vi "GetFormattedStringBounds.vi"(0 "reference":refnum<class "MultiLineString.lvclass">, 1 "graphics":refnum<class "Graphics.lvclass">, 5 "error in (no error)":errorcluster, 6 "TargetBounds(IgnoreIfZero)":T1 {"height" format="%.2f"; "width" format="%.2f"; "y" format="%.2f"; "x" format="%.2f"}) -> (14 "reference out":refnum<class "MultiLineString.lvclass">, 15 "bounds":T1 {"height" format="%.2f"; "width" format="%.2f"; "y" format="%.2f"; "x" format="%.2f"}, 19 "error out":errorcluster)   [LabVIEW 2020, in "MultiLineString.lvclass"]
doc: "public Rectangle2D getBounds(Graphics2D g2)"
uses:
  <resource>/Framework/Providers/Open_GDS/UML/MultiLineString_class/MultiLineString.lvclass
  <resource>/Framework/Providers/Open_GDS/UML/General/Rectangle/Rectangle Rectangle2D.ctl
  <resource>/Framework/Providers/Open_GDS/UML/Graphics_class/Graphics.lvclass
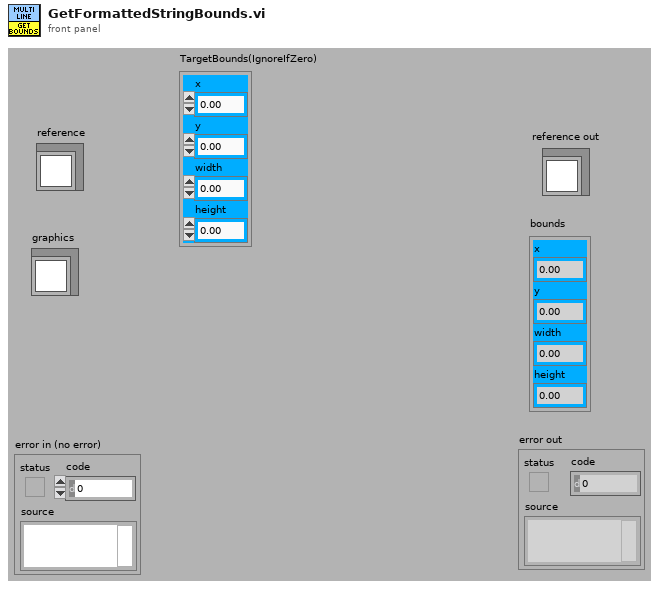
[diagram p1: front panel]
types:
  T1 = typedef "Rectangle Rectangle2D.ctl" = cluster{"x":dbl, "y":dbl, "width":dbl, "height":dbl}
  T2 = typedef "MultiLineString.lvclass/ObjectAttributes.ctl" = cluster{"GAP":i32, "text":string, "justification":T3, "size":T4, "underlined":bool}
  T3 = typedef "MultiLineString.lvclass/JustificationType.ctl" = enum16{"LEFT", "CENTER", "RIGHT"}
  T4 = typedef "MultiLineString.lvclass/SizeType.ctl" = enum16{"LARGE", "NORMAL", "SMALL"}
  T5 = typedef "Graphics.lvclass/FontType.ctl" = cluster{"Font Name:":string, "Size":i16, "Strikeout?":bool, "Italic?":bool, "Underline?":bool, "Outline?":bool, "Shadow?":bool, "Bold?":bool}
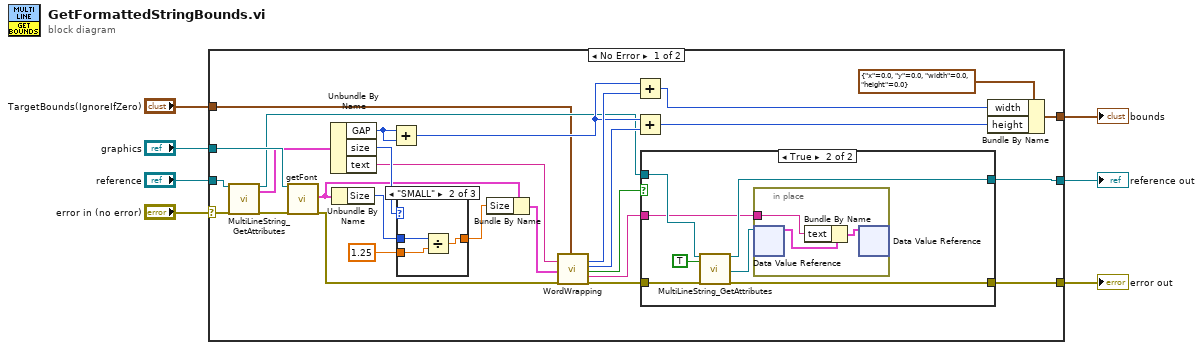
[diagram p0: block diagram]
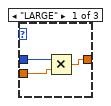
[diagram p3: hidden frame]
diagram:
  n1 = case shown="No Error" "error in (no error)" {
    selector: "error in (no error)" -> [w32 w55]
    tunnel: "reference" -> [w35 w56]
    tunnel: [w13 w55] -> w6
    tunnel: [w12 w56] -> w5
    tunnel: [w34 _] -> w3
    tunnel: "graphics" -> [w33 _]
    tunnel: "TargetBounds(IgnoreIfZero)" -> [w9 _]
    frame No Error {
      n2 = call <resource>:"MultiLineString_GetAttributes.vi"("reference in"=w35, "error in (no error)"=w32) -> ("reference out"=w15:refnum<class "MultiLineString.lvclass">, "Data"=w8:T2, "error out"=w19:errorcluster)  [unwired: 1 in, 14 out]
      n3 = call <resource>:"getFont.vi"("reference"=w33, "error in (no error)"=w19) -> ("font"=w28:T5, "error out"=w17:errorcluster)  [unwired: 16 out]
      n4 = Unbundle By Name(w8) -> ("GAP"=w26:i32, "size"=w29:T4, "text"=w24:string)
      n5 = Unbundle By Name(w28) -> ("Size"=w31:i16)
      n6 = Add(x=w26, y=w26) -> (x+y=w22:i32)
      n7 = case shown="\"SMALL\"" w29 {
        tunnel: w31 -> [w50 w52 w54]
        tunnel: 1.25 ("y") -> [w49 w53 _]
        tunnel: [w48 w51 w54] -> w27
        frame "LARGE" {
          n8 = Multiply(x=w50, y=w49) -> (x*y=w48:dbl)
        }
        frame "SMALL" {
          n9 = Divide(x=w52, y=w53) -> (x/y=w51:dbl)
        }
        frame "NORMAL", Default {
        }
      }
      n10 = Bundle By Name(cluster=w28, "Size"=w27) -> (w18:T5)
      n11 = call <resource>:"WordWrapping.vi"("FormattedMultiLineStringIn"=w24, "Font"=w18, "error in (no error)"=w17, "TargetBounds(IgnoreIfZero)"=w9) -> ("Width"=w23:i16, "Height"=w21:i16, "StringWrapped"=w10:bool, "WrappedFormattedMultiLineStringOut"=w11:string, "error out"=w14:errorcluster)  [unwired: 11 in]
      n12 = Add(x=w22, y=w23) -> (x+y=w25:i32)
      n13 = Add(x=w22, y=w21) -> (x+y=w20:i32)
      n14 = case shown="True" w10 {
        tunnel: w15 -> [w37 w44]
        tunnel: w14 -> [w36 w43]
        tunnel: [w36 w42] -> w13
        tunnel: [w37 w41] -> w12
        tunnel: w11 -> [_ w38]
        frame False {
        }
        frame True {
          n15 = call <resource>:"MultiLineString_GetAttributes.vi"("reference in"=w44, "OnlyGetDvrReference(False)"=TRUE, "error in (no error)"=w43) -> ("reference out"=w41:refnum<class "MultiLineString.lvclass">, "DataRef"=w39:refnum<data-value>, "error out"=w42:errorcluster)  [unwired: 13 in, 1 out]
          n16 = in-place {
            in-place-border: w38 -> [w46]
            n17 = in-place-dvr #1(w39) -> (w47:T2)  [unwired: 1 out]
            n18 = Bundle By Name(cluster=w47, "text"=w46) -> (w45:T2)
            n19 = in-place-dvr #1(w45) -> ()  [unwired: 2 out]
          }
        }
      }
      n20 = Bundle By Name(cluster=T1 {"x"=0.0, "y"=0.0, "width"=0.0, "height"=0.0} ("bounds"), "width"=w25, "height"=w20) -> (w34:T1)
    }
    frame Error {
    }
  }
  "reference out" <- w5
  "error out" <- w6
  "bounds" <- w3
